vi "Write Icon Data to Library.vi"(8 "error in":errorcluster, 10 "Data":string, 11 "Library Ref in":refnum<vi>) -> (0 "error out":errorcluster, 3 "Library Ref out":refnum<vi>)   [LabVIEW 2020, in "lv_icon.lvlib"]
doc: "Set the LabVIEW Icon Data of a Library."
uses:
  lv_icon.lvlib
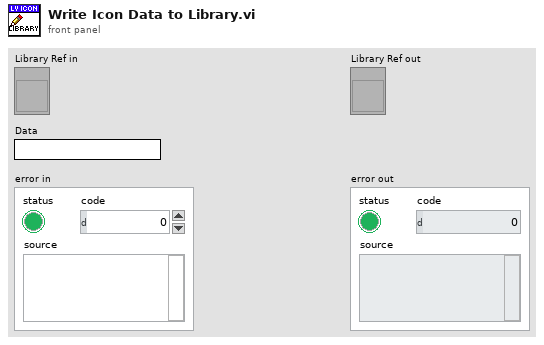
[diagram p1: front panel]
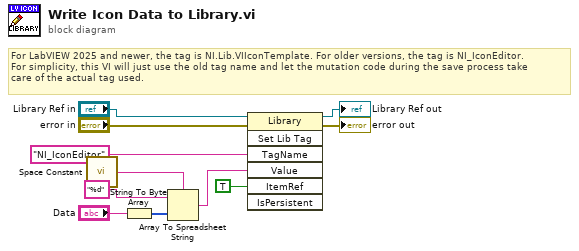
[diagram p0: block diagram]
diagram:
  # "For LabVIEW 2025 and newer, the tag is NI.Lib.VIIconTemplate. For older versions, the tag is NI_IconEditor.\nFor simplicity, this VI will just use the old tag name and let the mutation code during the save process take\ncare of the actual tag used."
  n1 = call <vilib>:"Space Constant.vi"() -> ("String"=w5:string)
  n2 = String To Byte Array(string="Data") -> (unsigned byte array=w8:u8[])
  n3 = Array To Spreadsheet String(delimiter (Tab)=w5, array=w8, 3:"%d" ("format string")) -> (spreadsheet string=w6:string)
  n4 = invoke class="Library" method="Set Lib Tag"(reference="Library Ref in", error in="error in", "TagName"="NI_IconEditor" ("Tag Name"), "Value"=w6, "ItemRef"=TRUE ("Is Persistent")) -> (reference out=→"Library Ref out":refnum<vi>, error out=→"error out":errorcluster)  [unwired: 2 in, 5 out]
